vi "Get Plugin Paths.vi"(8 "error in":errorcluster, 11 "measurement in":refnum<class "Continuous Counting Measurement.lvclass">) -> (0 "error out":errorcluster, 2 "plugin paths":T1, 3 "measurement out":refnum<class "Continuous Counting Measurement.lvclass">)   [LabVIEW 2021, in "MeasurementServerTests.lvlib" / "Measurement Service Tests.lvlib" / "Continuous Counting Measurement.lvclass"]
uses:
  Continuous Counting Measurement.lvclass
  Runtime/Measurements/Measurement Plugin Service/Plugin Paths.ctl
  _Get Type Specializations.vi
  _Get Measurement Details.vi
  _Measurement Logic.vi
  _Get UI Details.vi
  Measurement Configuration.ctl
  Measurement Results.ctl
  Runtime/Measurements/Measurement Plugin Service/Measurement Plugin Service.lvclass
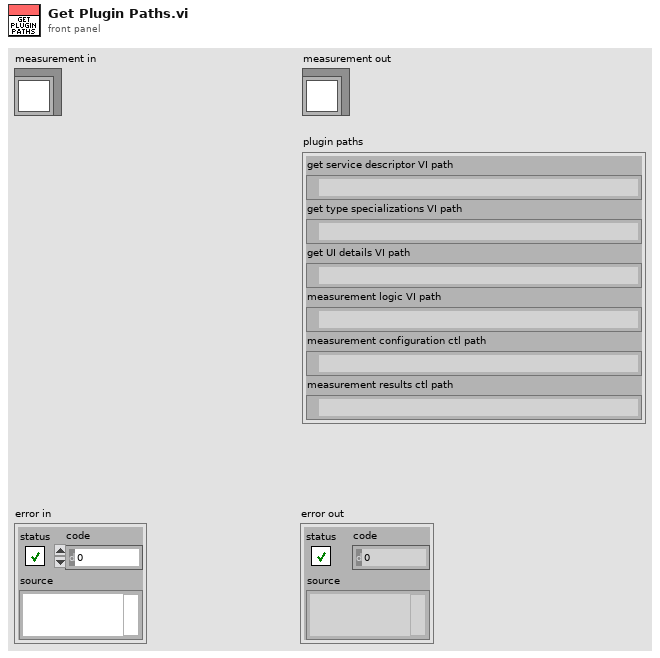
[diagram p1: front panel]
types:
  T1 = typedef "NI Measurement Plug-In SDK.lvlib/Measurement Plugin Service.lvclass/Plugin Paths.ctl" = cluster{"get service descriptor VI path":path, "get type specializations VI path":path, "get UI details VI path":path, "measurement logic VI path":path, "measurement configuration ctl path":path, "measurement results ctl path":path}
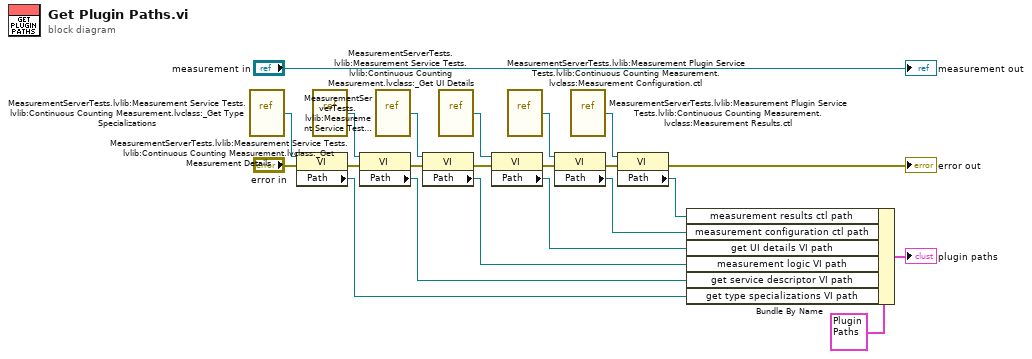
[diagram p0: block diagram]
diagram:
  n1 = vi-ref "MeasurementServerTests.lvlib:Measurement Service Tests.lvlib:Continuous Counting Measurement.lvclass:_Get Type Specializations.vi"() -> (w10:refnum<vi>)
  n2 = property class="VI"(reference=w10, error in="error in") -> (error out=w20:errorcluster, "Path"=w19:path)  [unwired: 1 out]
  n3 = vi-ref "MeasurementServerTests.lvlib:Measurement Service Tests.lvlib:Continuous Counting Measurement.lvclass:_Get Measurement Details.vi"() -> (w9:refnum<vi>)
  n4 = property class="VI"(reference=w9, error in=w20) -> (error out=w2:errorcluster, "Path"=w18:path)  [unwired: 1 out]
  n5 = vi-ref "MeasurementServerTests.lvlib:Measurement Service Tests.lvlib:Continuous Counting Measurement.lvclass:_Measurement Logic.vi"() -> (w8:refnum<vi>)
  n6 = property class="VI"(reference=w8, error in=w2) -> (error out=w4:errorcluster, "Path"=w3:path)  [unwired: 1 out]
  n7 = vi-ref "MeasurementServerTests.lvlib:Measurement Service Tests.lvlib:Continuous Counting Measurement.lvclass:_Get UI Details.vi"() -> (w7:refnum<vi>)
  n8 = property class="VI"(reference=w7, error in=w4) -> (error out=w22:errorcluster, "Path"=w17:path)  [unwired: 1 out]
  n9 = vi-ref "MeasurementServerTests.lvlib:Measurement Plugin Service Tests.lvlib:Continuous Counting Measurement.lvclass:Measurement Configuration.ctl"() -> (w5:refnum<vi>)
  n10 = property class="VI"(reference=w5, error in=w22) -> (error out=w21:errorcluster, "Path"=w16:path)  [unwired: 1 out]
  n11 = vi-ref "MeasurementServerTests.lvlib:Measurement Plugin Service Tests.lvlib:Continuous Counting Measurement.lvclass:Measurement Results.ctl"() -> (w6:refnum<vi>)
  n12 = property class="VI"(reference=w6, error in=w21) -> (error out=→"error out":errorcluster, "Path"=w15:path)  [unwired: 1 out]
  n13 = Bundle By Name(cluster=T1 {"get service descriptor VI path"=path "", "get type specializations VI path"=path "", "get UI details VI path"=path "", "measurement logic VI path"=path "", "measurement configuration ctl path"=path "", "measurement results ctl path"=path ""} ("plugin paths"), "measurement results ctl path"=w15, "measurement configuration ctl path"=w16, "get UI details VI path"=w17, "measurement logic VI path"=w3, "get service descriptor VI path"=w18, "get type specializations VI path"=w19) -> (→"plugin paths":T1)
  "measurement out" <- "measurement in"
